vi "Echo_Send_Echo_API.vi"(5 "frames":T5 {"flags" format="%.0x"; "id" format="%.0x"}, 6 "frame":T3 {"id" format="%.0x"}, 7 "context":T6 {"ack hi" format="%.0x"; "ack lo" format="%.0x"; "test hi" format="%.0x"; "test lo" format="%.0x"}, 8 "error in (no error)":errorcluster, 9 "counters in":T1, 10 "time store in":T2, 11 "channel in":refnum<class "CANsub_Channel.lvclass">) -> (0 "error out":errorcluster, 1 "counters out":T1, 2 "time store out":T2, 3 "channel out":refnum<class "CANsub_Channel.lvclass">)   [LabVIEW 2021]
doc: "S5 echo via API, Test case: Write_Echo of frame index at ID + echo offset (keeps IDE/FDF/BRS), time-stamped before and after with High Resolution Relative Seconds; stores t_dev, t_rx_lv, t_send_lv at key; echoes sent + 1. Loop-safe: no allocation, bounded time."
uses:
  api/CANsub_Channel/CANsub_Channel.lvclass
  Echo_Time_Store.ctl
  Echo_Counters.ctl
  Echo_Context.ctl
  Echo_Frame_Kind.ctl
  Echo_Frame.ctl
  api/Typedefs/CANsub_Frames.ctl
  api/CANsub_API.lvlib
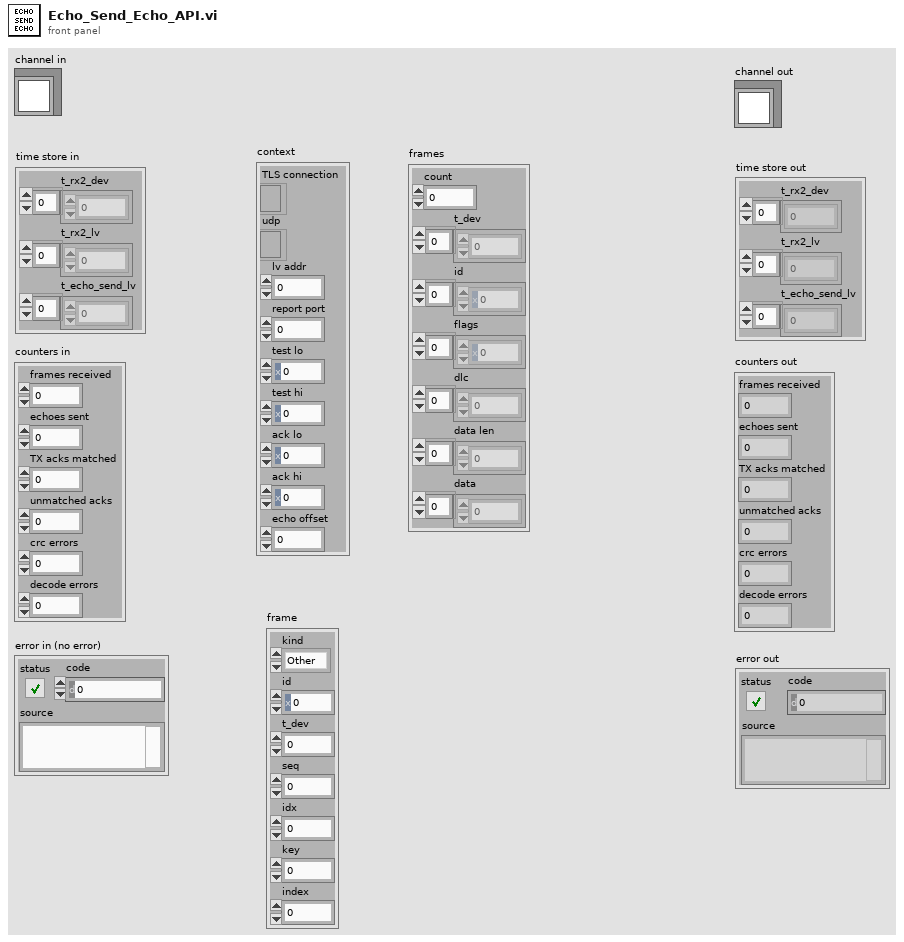
[diagram p1: front panel]
types:
  T1 = typedef "Echo_Counters.ctl" = cluster{"frames received":u32, "echoes sent":u32, "TX acks matched":u32, "unmatched acks":u32, "crc errors":u32, "decode errors":i32}
  T2 = typedef "Echo_Time_Store.ctl" = cluster{"t_rx2_dev":dbl[], "t_rx2_lv":dbl[], "t_echo_send_lv":dbl[]}
  T3 = typedef "Echo_Frame.ctl" = cluster{"kind":T4, "id":u32, "t_dev":dbl, "seq":u16, "idx":u8, "key":i32, "index":i32}
  T4 = typedef "Echo_Frame_Kind.ctl" = enum16{"Other", "Test", "Ack"}
  T5 = typedef "CANsub_API.lvlib/CANsub_Frames.ctl" = cluster{"count":i32, "t_dev":dbl[], "id":u32[], "flags":u16[], "dlc":u8[], "data len":u8[], "data":u8[]}
  T6 = typedef "Echo_Context.ctl" = cluster{"TLS connection":refnum<k5>, "udp":refnum<k16>, "lv addr":u32, "report port":u16, "test lo":u32, "test hi":u32, "ack lo":u32, "ack hi":u32, "echo offset":i32}
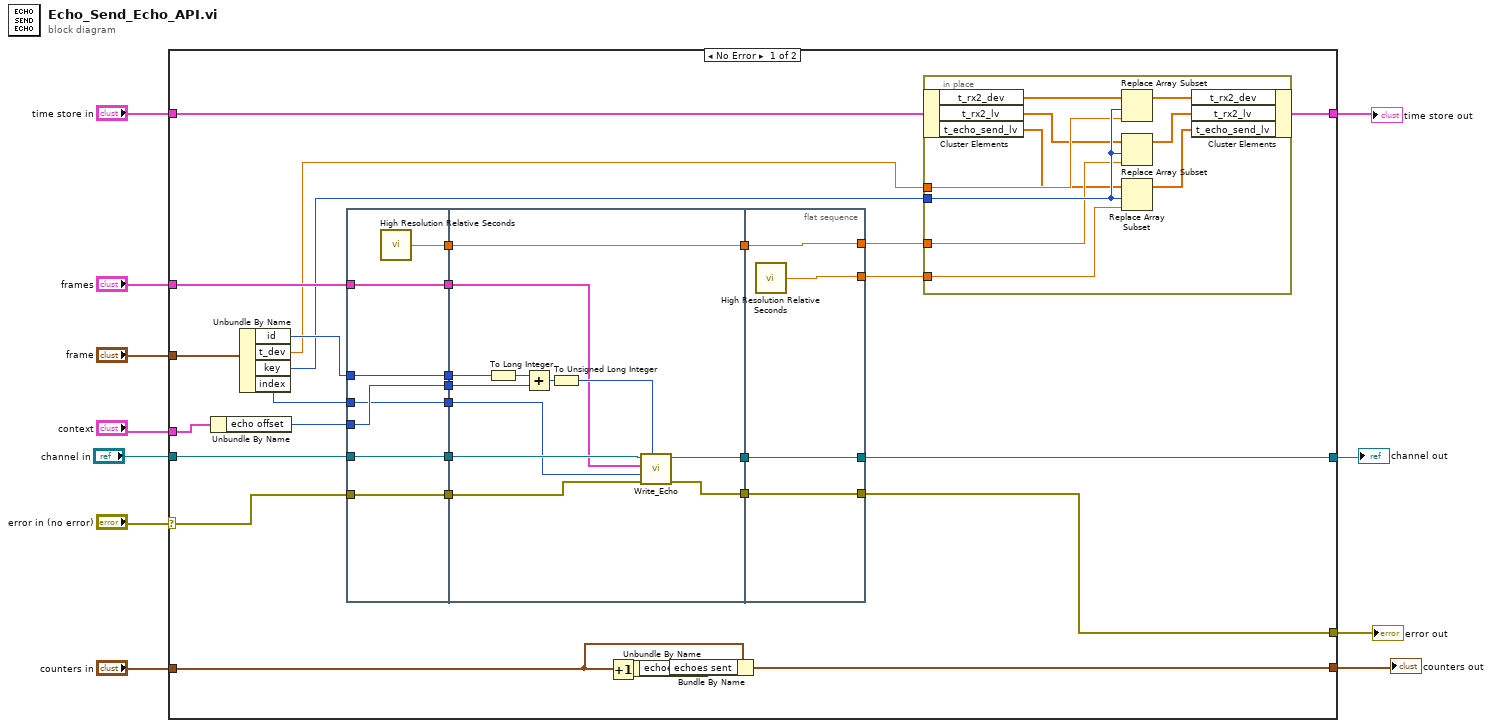
[diagram p0: block diagram]
diagram:
  n1 = case shown="No Error" "error in (no error)" {
    selector: "error in (no error)" -> [w28 w78]
    tunnel: [w16 w78] -> w10
    tunnel: [w21 w77] -> w9
    tunnel: "time store in" -> [w26 w77]
    tunnel: [w17 w76] -> w7
    tunnel: "counters in" -> [w19 w76]
    tunnel: "frame" -> [w40 _]
    tunnel: "context" -> [w39 _]
    tunnel: "frames" -> [w30 _]
    tunnel: "channel in" -> [w14 w75]
    tunnel: [w12 w75] -> w1
    frame No Error {
      n2 = Unbundle By Name(w39) -> ("echo offset"=w34:i32)
      n3 = Unbundle By Name(w40) -> ("id"=w37:u32, "t_dev"=w25:dbl, "key"=w24:i32, "index"=w33:i32)
      n4 = flat-sequence {
        tunnel: [w48] -> w41
        tunnel: w37 -> [w47]
        tunnel: [w47] -> w36
        tunnel: [w46] -> w35
        tunnel: w34 -> [w46]
        tunnel: w33 -> [w45]
        tunnel: [w45] -> w32
        tunnel: [w44] -> w31
        tunnel: w30 -> [w44]
        tunnel: [w43] -> w29
        tunnel: w28 -> [w43]
        tunnel: [w42] -> w15
        tunnel: w14 -> [w42]
        tunnel: w41 -> [w60]
        tunnel: [w60] -> w38
        tunnel: w36 -> [w59]
        tunnel: w35 -> [w57]
        tunnel: w32 -> [w50]
        tunnel: w31 -> [w51]
        tunnel: w29 -> [w49]
        tunnel: [w53] -> w27
        tunnel: w15 -> [w55]
        tunnel: [w54] -> w13
        tunnel: [w64] -> w22
        tunnel: w38 -> [w64]
        tunnel: [w63] -> w23
        tunnel: [w62] -> w16
        tunnel: w27 -> [w62]
        tunnel: [w61] -> w12
        tunnel: w13 -> [w61]
        frame #0 {
          n5 = call <vilib>:"High Resolution Relative Seconds.vi"() -> ("relative seconds"=w48:dbl)
        }
        frame #1 {
          n6 = To Long Integer(number=w59) -> (32bit integer=w58:i32)
          n7 = Add(x=w58, y=w57) -> (x+y=w56:i32)
          n8 = To Unsigned Long Integer(number=w56) -> (unsigned 32bit integer=w52:u32)
          n9 = call-dynamic "Write_Echo.vi"("new id"=w52, "error in (no error)"=w49, "i"=w50, "frames"=w51, "channel in"=w55) -> ("error out"=w53:errorcluster, "channel out"=w54:refnum<class "CANsub_Channel.lvclass">)  [unwired: 5 in]
        }
        frame #2 {
          n10 = call <vilib>:"High Resolution Relative Seconds.vi"() -> ("relative seconds"=w63:dbl)
        }
      }
      n11 = Unbundle By Name(w19) -> ("echoes sent"=w20:u32)
      n12 = Increment(x=w20) -> (x+1=w18:u32)
      n13 = Bundle By Name(cluster=w19, "echoes sent"=w18) -> (w17:T1)
      n14 = in-place {
        in-place-border: w25 -> [w72]
        in-place-border: w24 -> [w74]
        in-place-border: w23 -> [w73]
        in-place-border: w22 -> [w71]
        n15 = in-place-cluster #1(w26) -> ("t_rx2_dev"=w70:dbl[], "t_rx2_lv"=w69:dbl[], "t_echo_send_lv"=w68:dbl[])
        n16 = Replace Array Subset(array=w70, new element=w72, index=w74) -> (w67:dbl[])
        n17 = Replace Array Subset(array=w69, new element=w71, index=w74) -> (w66:dbl[])
        n18 = Replace Array Subset(array=w68, new element=w73, index=w74) -> (w65:dbl[])
        n19 = in-place-cluster #1("t_rx2_dev"=w67, "t_rx2_lv"=w66, "t_echo_send_lv"=w65) -> (w21:T2)
      }
    }
    frame Error {
    }
  }
  "time store out" <- w9
  "counters out" <- w7
  "error out" <- w10
  "channel out" <- w1
